vi "Update SyncMethod Event Structure.vi"(7 "gRPC Method Parameters":T1[](array[typedef]), 8 "error in (no error)":errorcluster, 10 "Newly created methods count":i64, 11 "Server class in":refnum<vi>) -> (0 "error out":errorcluster, 3 "Server class out":refnum<vi>)   [LabVIEW 2019, in "gRPC Template Creation Utility.lvlib"]
uses:
  gRPC Template Creation Utility.lvlib
  TypeDefs/RPC Method Parameters.ctl
  <vilib>/event_ctls.llb/lveventtype.ctl
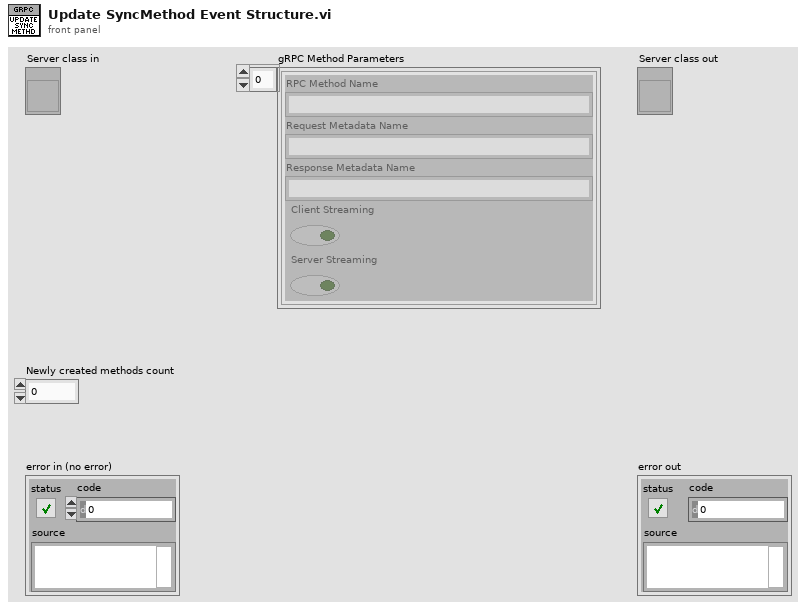
[diagram p1: front panel]
types:
  T1 = typedef "gRPC Template Creation Utility.lvlib/RPC Method Parameters.ctl" = cluster{"RPC Method Name":string, "Request Metadata Name":string, "Response Metadata Name":string, "Client Streaming":bool, "Server Streaming":bool}
  T2 = typedef "lveventtype.ctl" = enum32{"Null", "Timeout", "Annotation Menu Selection", "Annotation Menu Selection?", "App Instance Close", "App Instance Close?", "Autoscale Range Change", "Bookmark Info Change", "Cell Edit", "Cell Edit?", "Cursor Grab", "Cursor Grab?", "Cursor Menu Selection", "Cursor Menu Selection?", "Cursor Move", "Cursor Release", "Data Change", "Direction Change", "Display State Change", "Drag Ended", "Drag Enter", "Drag Leave", "Drag Over", "Drag Source Update", "Drag Starting", "Drag Starting?", "Drop", "Exec State Change", "Key Down", "Key Down?", "Key Repeat", "Key Repeat?", "Key Up", "Listbox Double Click", "Menu Activation?", "Menu Selection (App)", "Menu Selection? (App)", "Menu Selection (User)", "Mouse Down", "Mouse Down?", "Mouse Enter", "Mouse Leave", "Mouse Move", "Mouse Up", "Mouse Wheel", "NI Security User Change (App)", "Pane Size", "Panel Close", "Panel Close?", "Panel Resize", "Plot Attribute Change", "Scale Range Change", "Shortcut Menu Activation?", "Shortcut Menu Selection (App)", "Shortcut Menu Selection? (App)", "Shortcut Menu Selection (User)", "Tree Double Click", "Tree Drag", "Tree Drag?", "Tree Drop", "Tree Drop?", "Tree Item Close", "Tree Item Close?", "Tree Item Open", "Tree Item Open?", "User Event", "Value Change"}
  T3 = cluster{"Event Type":T2, "Event Registration Index":i32}
  T4 = cluster{"Event Type":T2, "Event Registration Index":i32}[]
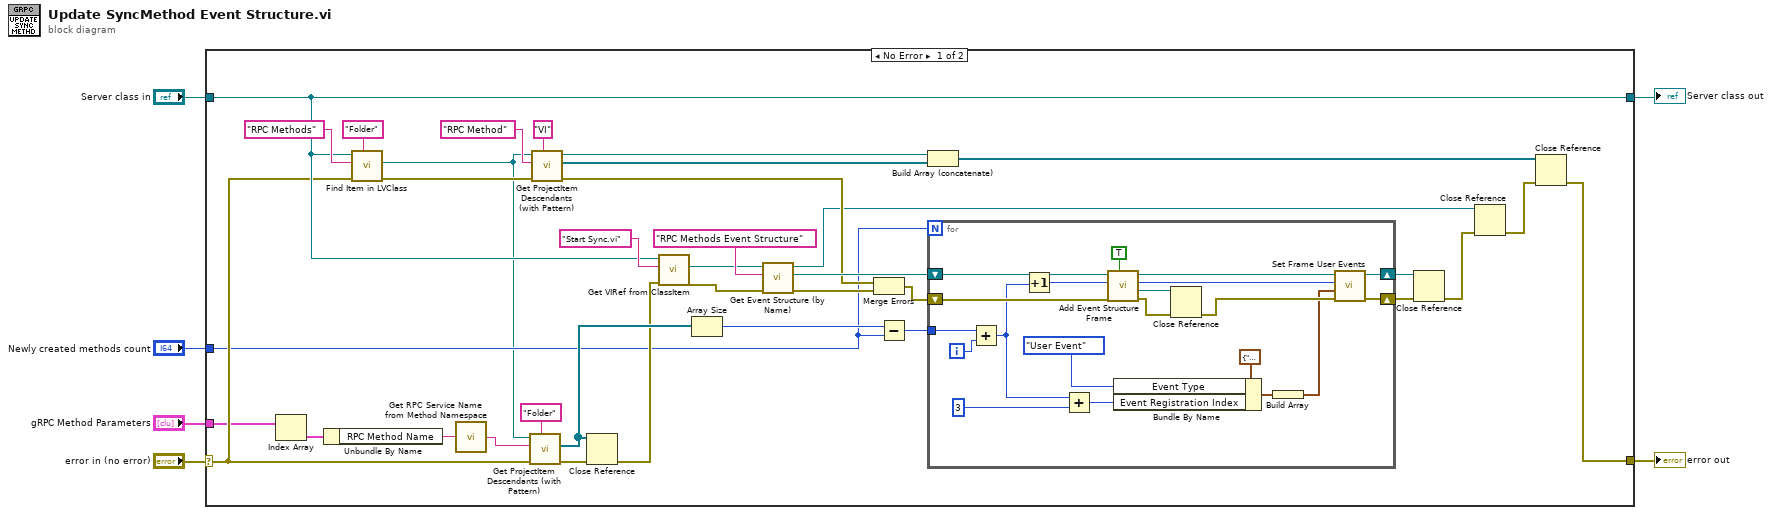
[diagram p0: block diagram]
diagram:
  n1 = case shown="No Error" "error in (no error)" {
    selector: "error in (no error)" -> [w15 w63]
    tunnel: "Server class in" -> [w20 w64]
    tunnel: [w21 w63] -> w5
    tunnel: [w20 w64] -> w3
    tunnel: "Newly created methods count" -> [w9 _]
    tunnel: "gRPC Method Parameters" -> [w14 _]
    frame No Error {
      n2 = Index Array(array=w14) -> (element=w19:T1)  [unwired: 1 in]
      n3 = Unbundle By Name(w19) -> ("RPC Method Name"=w18:string)
      n4 = call "Find Item in LVClass.vi"("Item Type"="Folder", "error in (no error)"=w15, "Item Name"="RPC Methods", "Class Item in"=w20) -> ("error out"=w42:errorcluster, "Project Item (Class Item)"=w7:refnum<vi>)  [unwired: 4 in, 2 out]
      n5 = call "Get RPC Service Name from Method Namespace.vi"("RPC Method Name"=w18) -> ("RPC Service Name"=w17:string)
      n6 = call "Get ProjectItem Descendants (with Pattern).vi"("Type"="Folder", "error in (no error)"=w15, "Pattern"=w17, "ProjectItem in"=w7) -> ("error out"=w13:errorcluster, "ProjectItem descendents"=w12:refnum<vi>[])  [unwired: 5 in, 1 out]
      n7 = call "Get ProjectItem Descendants (with Pattern).vi"("Type"="VI", "error in (no error)"=w42, "Pattern"="RPC Method" ("regular expression"), "ProjectItem in"=w7) -> ("error out"=w27:errorcluster, "ProjectItem descendents"=w25:refnum<vi>[], "ProjectItem out"=w30:refnum<vi>)  [unwired: 5 in]
      n8 = Close Reference(reference=w12, error in (no error)=w13) -> (error out=w11:errorcluster)
      n9 = call "Get VIRef from ClassItem.vi"("error in (no error)"=w11, "Item Name"="Start Sync.vi", "LVClassLibrary in"=w20) -> ("error out"=w34:errorcluster, "VIref out"=w36:refnum<vi>)  [unwired: 5 in, 2 out]
      n10 = Array Size(array=w12) -> (size(s)=w10:i32)
      n11 = call "Get Event Structure (by Name).vi"("error in (no error)"=w34, "Label"="RPC Methods Event Structure", "Owner VI in"=w36) -> ("error out"=w28:errorcluster, "Event Structure ref out"=w33:refnum<vi>, "Owner VI out"=w23:refnum<vi>)  [unwired: 5 in, 1 out]
      n12 = Merge Errors(w27, w28) -> (w26:errorcluster)
      n13 = Subtract(x=w10, y=w9) -> (x-y=w8:i64)
      n14 = Build Array (concatenate)(w30, w25) -> (w29:refnum<vi>[])
      n15 = for {
        N: w9 -> [_]
        shift-right: [w49] -> w32
        shift-left: w26 -> [w47]
        shift-right: [w46] -> w31
        shift-left: w33 -> [w48]
        tunnel: w8 -> [w44]
        i -> [w45]
        n16 = Add(x=w44, y=w45) -> (x+y=w43:i64)
        n17 = Increment(x=w43) -> (x+1=w56:i64)
        n18 = Add(x=w43, y=3) -> (x+y=w52:i64)
        n19 = call "Add Event Structure Frame.vi"("After? (T)"=TRUE, "error in (no error)"=w47, "Reference Frame Index"=w56, "Event Structure ref in"=w48) -> ("error out"=w62:errorcluster, "Added Frame"=w61:refnum<vi>, "Added Frame Index"=w59:i32, "Event Structure ref out"=w58:refnum<vi>)  [unwired: 4 in]
        n20 = Bundle By Name(cluster=T3 {"Event Type"=enum."User Event", "Event Registration Index"=3} ("Dynamic Events"), "Event Type"=lveventtype."User Event", "Event Registration Index"=w52) -> (w51:T3)
        n21 = Close Reference(reference=w61, error in (no error)=w62) -> (error out=w60:errorcluster)
        n22 = Build Array(w51) -> (w50:T4)
        n23 = call "Set Frame User Events.vi"("error in (no error)"=w60, "Dynamic Events"=w50, "Frame Index in"=w59, "Event Structure ref in"=w58) -> ("error out"=w49:errorcluster, "Event Structure ref out"=w46:refnum<vi>)  [unwired: 5 in, 1 out]
      }
      n24 = Close Reference(reference=w31, error in (no error)=w32) -> (error out=w24:errorcluster)
      n25 = Close Reference(reference=w23, error in (no error)=w24) -> (error out=w22:errorcluster)
      n26 = Close Reference(reference=w29, error in (no error)=w22) -> (error out=w21:errorcluster)
    }
    frame Error {
    }
  }
  "error out" <- w5
  "Server class out" <- w3
